vi "The Need for JTFA.vi"() -> ()   [LabVIEW 2019]
doc: "This example shows the circumstances under which you need time-frequency analysis. For a nonstationary signal, the Fourier transform-based power spectrum may provide useless information or even misleading information. This example illustrates two linear chirp signals. Each signal is a time-reversed version of the other. The power spectrum of the two signals show no differences, while the time-varying frequency contents of the two signals are indicated clearly in the spectrograms.\n\n<b>Instructions:</b>\n1) Run this VI.\n2) Compare the power spectrum and spectrogram of the two signals. Notice how the power spectra are identical, while the spectrograms are different due to the time-varying frequency components."
uses:
  <vilib>/Analysis/4window.llb/windowTd.ctl
  <vilib>/addons/Time Frequency Analysis/typedefs.llb/TFA Data.ctl
  Instance           5 25Saved   The Need for JTFA .vi
  <vilib>/measure/maspectr.llb/FFT Power Spectrum and PSD for 1 Chan.vi
  <vilib>/addons/Time Frequency Analysis/_control.llb/TFA Configure Spectrogram Indicator (Predefined Color Table).vi
  <vilib>/addons/_Advanced Signal Processing/NI_AdvSigProcTFA.lvlib
  <vilib>/Analysis/NI_AALPro.lvlib
  <vilib>/measure/NI_MAPro.lvlib
panel:
  out "size(s) 2":i32
  out "size(s)":i32[](array[numeric])
  in  "Horizontal Pointer Slide":dbl(slide) scale=0.0..1.0
  out "Waveform Graph":T1(graph)
  in  "Stop":bool
  out "Mean Frequency":cluster{"f0":dbl, "df":dbl, "S(f)":dbl[]}(graph)
  in  "trimmed percent":cluster{"upper":dbl, "lower":dbl} {"lower" min=0.0 max=100.0 format="%#_g %"; "upper" min=0.0 max=100.0 format="%#_g %"}
  in  "File Path Control":path=path "\\\\eden\\NHMFLDATA/Data/cell3daq/January_2020/012820/p012_012820.tdms"
  out "aspt-left-top":bool
  out "Power Spectrum of the Linear Chirp":cluster{"f0":dbl, "df":dbl, "magnitude":dbl[]}(graph)
  out "Spectrogram of the Linear Chirp":dbl[][](graph)
  out "Linear Chirp":waveform(dbl)(graph)
  # "Overview: Shows the circumstances under which you need time-frequency analysis. \nRequirements: LabVIEW Full Development System, Advanced Signal Processing Toolkit\nInstructions: \n1. Run this VI.\n2. Compare the power spectrum and spectrogram of the two signals. Notice how the power spectra are identical, while the spectrograms are different due to the time-varying frequency components."
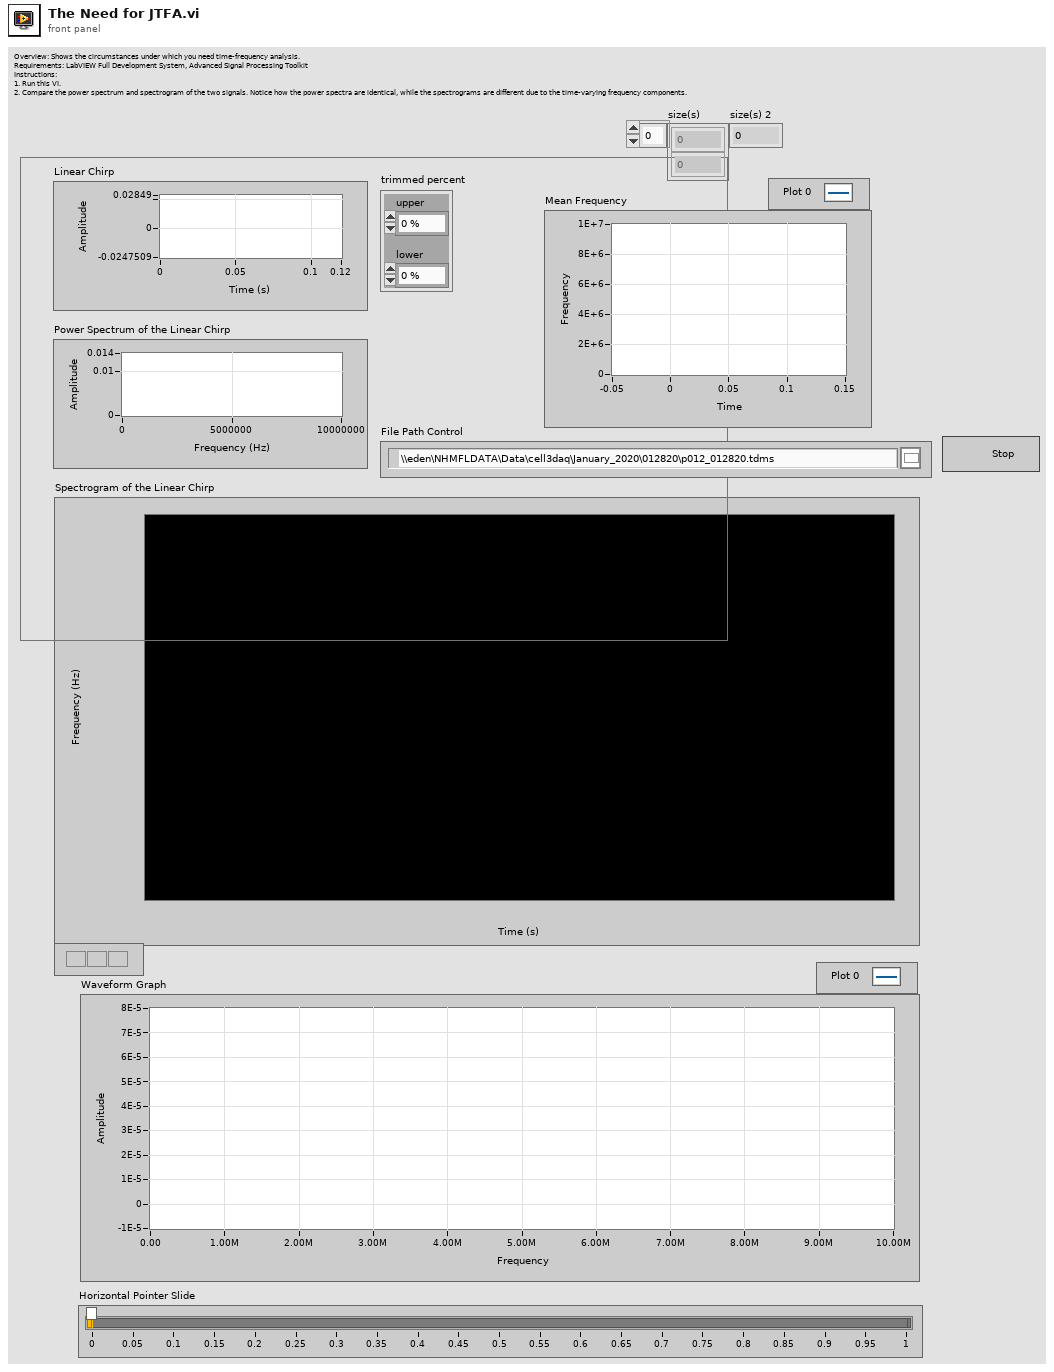
[diagram p1: front panel]
types:
  T1 = cluster{"frequency offset":dbl, "frequency multiplier":dbl, "Spectrogram":dbl[]}
  T2 = typedef "NI_AALPro.lvlib/windowTd.ctl" = u32
  T3 = typedef "NI_AdvSigProcTFA.lvlib/TFA Data.ctl" = u16
  T4 = cluster{"frequency offset":dbl, "frequency multiplier":dbl}
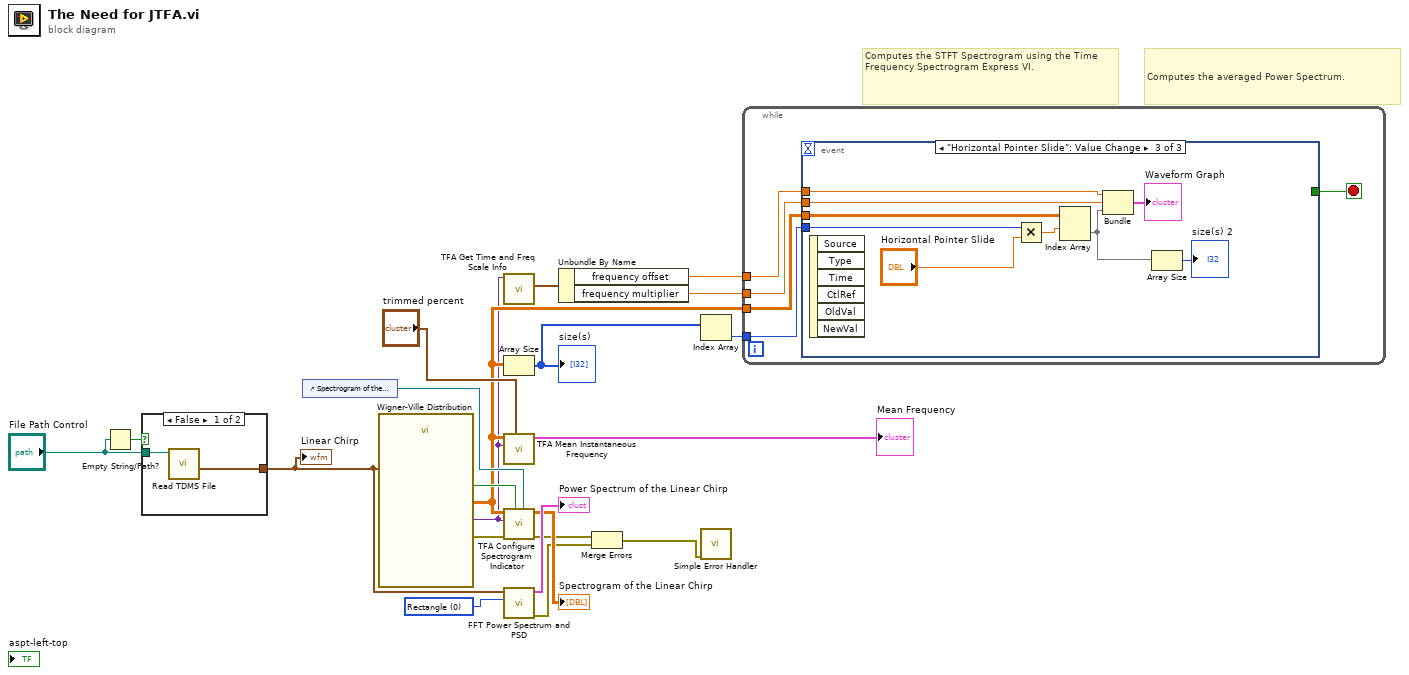
[diagram p0: block diagram]
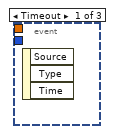
[diagram p2: hidden frame]
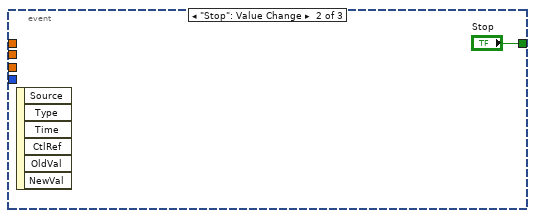
[diagram p3: hidden frame]
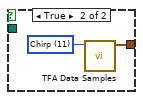
[diagram p4: hidden frame]
diagram:
  w16 = T2 0 items=["Rectangle"=0, "Hanning"=1, "Hamming"=2, "Blackman-Harris"=3, "Exact Blackman"=4, "Blackman"=5, "Flat Top"=6, "4 Term B-Harris "=7, "7 Term B-Harris"=8, "Low Sidelobe"=9, "Blackman Nuttall"=11, "Triangle"=30, "Bartlett-Hanning"=31, "Bohman"=32, "Parzen"=33, "Welch"=34, "Kaiser"=60, "Dolph-Chebyshev"=61, "Gaussian"=62] ("window")
  # "Computes the averaged Power Spectrum."
  # "Computes the STFT Spectrogram using the Time Frequency Spectrogram Express VI."
  n1 = Empty String/Path?(string/path="File Path Control") -> (empty?=w10:bool)
  n2 = case shown="False" w10 {
    tunnel: [w23 w25] -> w18
    tunnel: "File Path Control" -> [w22 _]
    frame False {
      n3 = call "Read TDMS File.vi"("File Path Control"=w22) -> ("Waveform"=w23:waveform(dbl))  [unwired: 8 in, 2 out]
    }
    frame True {
      w24 = T3 11 items=["PC Fan"=0, "Noisy Chirps"=1, "TDR 1"=2, "TDR 2"=3, "Liquefaction"=4, "Liquefaction Free"=5, "Aneurysm"=6, "Bat"=7, "RF"=8, "Two Gaussian"=9, "Three Gaussian"=10, "Chirp"=11, "Gaussian Chirp"=12, "Cross Chirp"=13, "Doppler"=14, "HOP"=15, "TF Sine"=16, "Three Tone"=17, "Four Tone"=23, "Blood Flow Doppler (phase a)"=20, "Blood Flow Doppler (phase b)"=21, "Heart sound"=22, "-"=18, "Random Noise"=19] ("data")
      n4 = call <vilib>:"TFA Data Samples.vi"("data"=w24) -> ("signal"=w25:waveform(dbl))  [unwired: 10 out]
    }
  }
  "Linear Chirp" <- w18
  n5 = control-ref of="Spectrogram of the Linear Chirp"() -> (w20:refnum<vi>)
  n6 = call "Wigner-Ville Distribution"("Signal"=w18) -> ("error out"=w15:errorcluster, "Scale Info"=w4:variant, "Spectrogram"=w5:dbl[][], "dB"=w17:bool)  [unwired: 2 in, 5 out]
  n7 = call <vilib>:"TFA Get Time and Freq Scale Info.vi"("scale info"=w4) -> ("frequency info"=w3:T4)  [unwired: 8 in, 2 out]
  n8 = Array Size(array=w5) -> (size(s)=w7:i32[])
  "size(s)" <- w7
  n9 = call <vilib>:"TFA Mean Instantaneous Frequency.vi"("trimmed percent"="trimmed percent", "scale info"=w4, "spectrogram"=w5) -> ("MIF"=→"Mean Frequency":cluster{"t0":dbl, "dt":dbl, "frequency":dbl[]})  [unwired: 7 in, 1 out]
  n10 = call-poly <vilib>:"TFA Configure Spectrogram Indicator.vi"("reference of TF spectrogram indicator"=w20, "dB on? (F)"=w17, "error in (no error)"=w15, "scale info"=w4, "spectrogram"=w5) -> ("error out"=w14:errorcluster, "TF spectrogram indicator"=→"Spectrogram of the Linear Chirp":dbl[][])  [unwired: 2 in, 3 out]
  n11 = call-poly <vilib>:"FFT Power Spectrum and PSD.vi"("window"=w16, "time signal"=w18) -> ("error out"=w13:errorcluster, "Power Spectrum / PSD"=→"Power Spectrum of the Linear Chirp":cluster{"f0":dbl, "df":dbl, "magnitude":dbl[]})  [unwired: 6 in, 2 out]
  n12 = Unbundle By Name(w3) -> ("frequency offset"=w2:dbl, "frequency multiplier"=w1:dbl)
  n13 = Merge Errors(w14, w13) -> (w12:errorcluster)
  n14 = Index Array(array=w7) -> (element=w6:i32)  [unwired: 1 in]
  n15 = call <vilib>:"Simple Error Handler.vi"("error in (no error)"=w12) -> ()  [unwired: 4 in, 5 out]
  n16 = while {
    tunnel: w6 -> [w29]
    tunnel: w5 -> [w28]
    tunnel: w2 -> [w27]
    tunnel: w1 -> [w26]
    stop <- w30 stop-if-true
    n17 = event shown="[2] \"Horizontal Pointer Slide\": Value Change" {
      selector: _ -> [_ _ _]
      dyn-events: _ -> [_ _ _]
      timeout: _ -> [_ _ _]
      tunnel: [_ "Stop" _] -> w30
      tunnel: w29 -> [_ _ w39]
      tunnel: w28 -> [_ _ w38]
      tunnel: w27 -> [_ _ w36]
      tunnel: w26 -> [_ _ w35]
      event Timeout {
        n18 = event-data() -> ()  [unwired: 1 in, 3 out]
      }
      event "Stop": Value Change {
        n19 = event-data() -> ()  [unwired: 1 in, 6 out]
      }
      event "Horizontal Pointer Slide": Value Change {
        n20 = event-data() -> ()  [unwired: 1 in, 6 out]
        n21 = Multiply(x=w39, y="Horizontal Pointer Slide") -> (x*y=w37:dbl)
        n22 = Index Array(array=w38, index (row)=w37) -> (element=w33:dbl[])  [unwired: 1 in]
        n23 = Bundle("frequency offset"=w36, "frequency multiplier"=w35, "Spectrogram"=w33) -> (→"Waveform Graph":T1)  [unwired: 1 in]
        n24 = Array Size(array=w33) -> (size(s)=→"size(s) 2":i32)
      }
    }
  }
